vi "New.vi"(8 "error in (no error)":errorcluster, 11 "ChannelMap":map{string, refnum<data-value>}(c390)) -> (0 "error out":errorcluster, 3 "plot handle":refnum<class "NIringPlotHandle.lvclass">)   [LabVIEW 2021, in "NIringPlotHandle.lvclass"]
uses:
  NIringPlotHandle.lvclass
  <vilib>/National Instruments/Variant Ring Buffer/Ring Buffer.lvclass
  NIringPlotHandle.lvclass/NIringPlotHandle.ctl
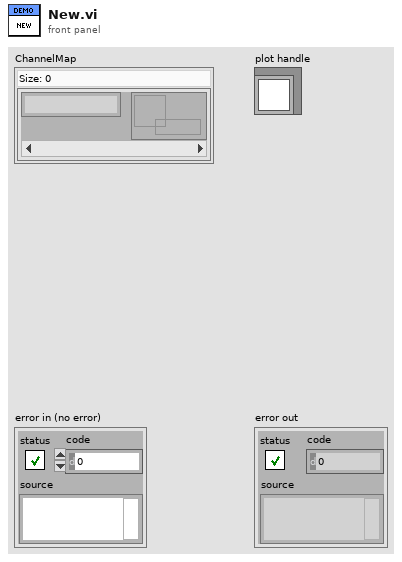
[diagram p1: front panel]
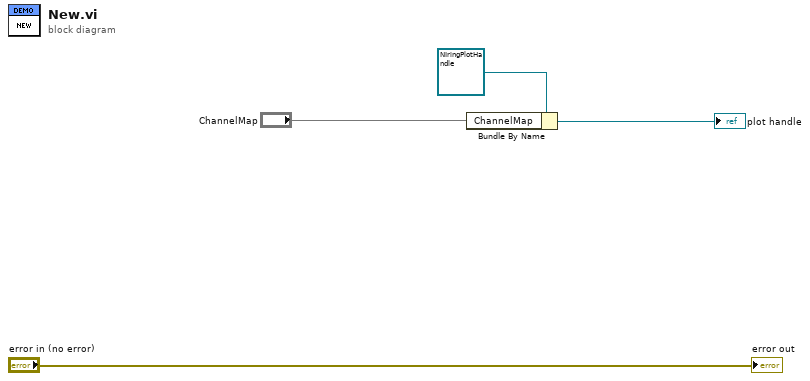
[diagram p0: block diagram]
diagram:
  n1 = Bundle By Name(cluster=refnum<class "NIringPlotHandle.lvclass"> refnum ("BluePlotDemo.lvlib:BluePlotHandleDemo.lvclass"), "ChannelMap"="ChannelMap") -> (→"plot handle":refnum<class "NIringPlotHandle.lvclass">)
  "error out" <- "error in (no error)"
